vi "Parse.vi"(10 "命令":string) -> (0 "结果字符串":string, 1 "数字":dbl, 2 "成功？":bool)   [LabVIEW 2026, in "UI-Zolix.lvlib"]
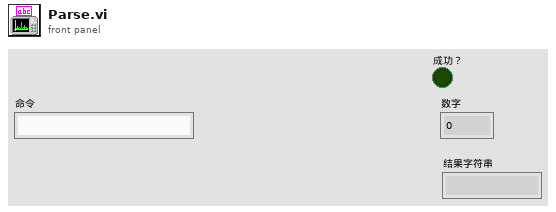
[diagram p1: front panel]
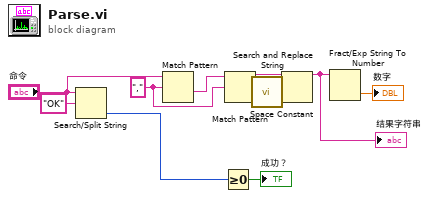
[diagram p0: block diagram]
diagram:
  w6 = "," ("搜索字符串/字符(-)")
  n1 = Search/Split String(string="命令", search string/char (-)="OK" ("搜索字符串/字符(-)")) -> (offset of match=w9:i32)  [unwired: 1 in, 2 out]
  n2 = Match Pattern(string="命令", regular expression=w6) -> (after substring=w5:string)  [unwired: 1 in, 3 out]
  n3 = Greater Or Equal To 0?(x=w9) -> (x >= 0?=→"成功？":bool)
  n4 = Match Pattern(string=w5, regular expression=w6) -> (before substring=w3:string)  [unwired: 1 in, 3 out]
  n5 = call <vilib>:"Space Constant.vi"() -> ("String"=w4:string)
  n6 = Search and Replace String(input string=w3, search string=w4) -> (result string=w1:string)  [unwired: 6 in, 3 out]
  "结果字符串" <- w1
  n7 = Fract/Exp String To Number(string=w1) -> (number=→"数字":dbl)  [unwired: 3 in, 1 out]
